vi "Parse Change TeraTerm Ant Pol.vi"(8 "error in (no error)":errorcluster caption="에러 입력(에러 없음)", 10 "JSON string":string, 11 "Instrument Manager 입력":refnum<class "Instrument Manager.lvclass">) -> (0 "error out":errorcluster caption="에러 출력", 1 "Antenna Pol":enum16{"H", "V"}(ring), 2 "Change TeraTerm Ant Pol Param":T1, 3 "Instrument Manager 출력":refnum<class "Instrument Manager.lvclass">)   [LabVIEW 2023, in "Instrument Manager.lvclass"]
uses:
  Instrument Manager.lvclass
  Instrument Manager.lvclass/Instrument Manager.ctl
  Param Definition/Change TeraTerm Ant Pol Param.ctl
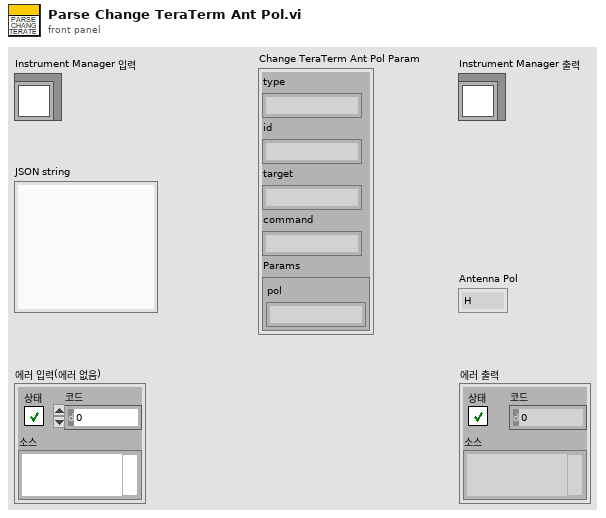
[diagram p1: front panel]
types:
  T1 = typedef "Instrument Manager.lvclass/Change TeraTerm Ant Pol Param.ctl" = cluster{"type":string, "id":string, "target":string, "command":string, "Params":cluster{"pol":string}}
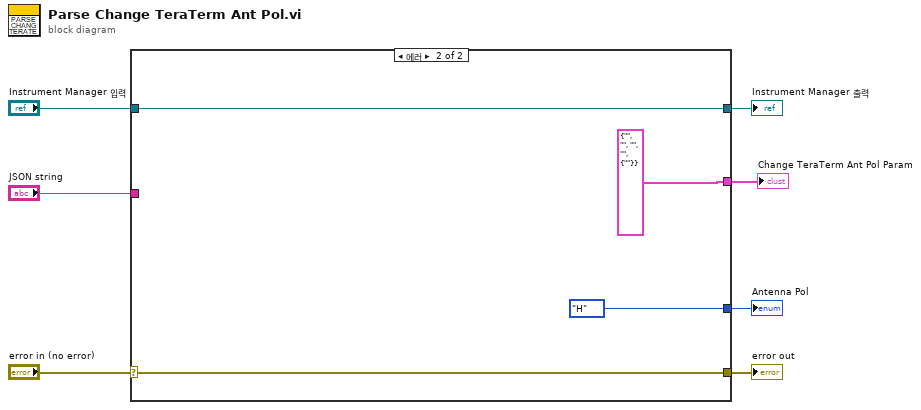
[diagram p0: block diagram]
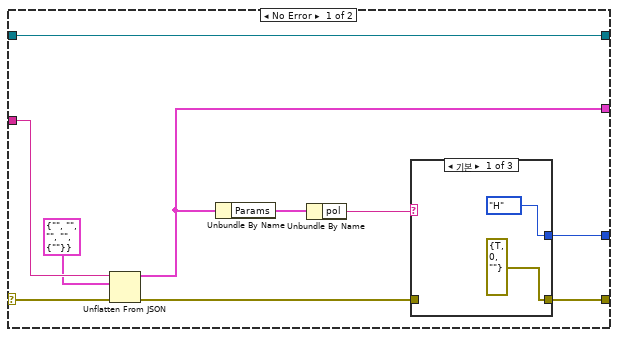
[diagram p2: hidden frame]
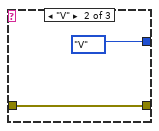
[diagram p3: hidden frame]
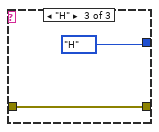
[diagram p4: hidden frame]
diagram:
  n1 = case shown="에러" "error in (no error)" {
    selector: "error in (no error)" -> [w15 w27]
    tunnel: [w14 w27] -> w6
    tunnel: [w17 w26] -> w4
    tunnel: "Instrument Manager 입력" -> [w17 w26]
    tunnel: "JSON string" -> [w13 _]
    tunnel: [w12 enum16{"H", "V"}."H" ("Antenna Pol")] -> w2
    tunnel: [w8 T1 {"type"="", "id"="", "target"="", "command"="", "Params"={"pol"=""}} ("Change TeraTerm Ant Pol Param")] -> w1
    frame No Error {
      n2 = Unflatten From JSON(JSON string=w13, type and defaults=T1 {"type"="", "id"="", "target"="", "command"="", "Params"={"pol"=""}} ("Change TeraTerm Ant Pol Param"), error in (no error)=w15) -> (value=w8:T1, error out=w16:errorcluster)  [unwired: 4 in]
      n3 = Unbundle By Name(w8) -> ("Params"=w11:cluster{"pol":string})
      n4 = Unbundle By Name(w11) -> ("pol"=w10:string)
      n5 = case shown="기본" w10 {
        tunnel: w16 -> [_ w21 w22]
        tunnel: [errorcluster {"status"=TRUE, "code"=0, "source"=""} ("error out") w21 w22] -> w14
        tunnel: [enum16{"H", "V"}."H" ("Antenna Pol") enum16{"H", "V"}."V" ("Antenna Pol") enum16{"H", "V"}."H" ("Antenna Pol")] -> w12
        frame Default {
        }
        frame "V" {
        }
        frame "H" {
        }
      }
    }
    frame Error {
    }
  }
  "error out" <- w6
  "Instrument Manager 출력" <- w4
  "Antenna Pol" <- w2
  "Change TeraTerm Ant Pol Param" <- w1
